vi "Parse Request-JSONtext.vi"(8 "error in (no error)":errorcluster, 10 "<JSON> Request":string) -> (0 "error out":errorcluster, 1 "params":string, 2 "method":string, 4 "id":string)   [LabVIEW 2019, in "JSON-RPC.lvlib"]
uses:
  JSON-RPC.lvlib
  66b5d778-a0b8-403e-b727-bb36a32d382a.vi
  6814ee06-2257-4c2f-8f04-31d91309bef7.vi
  f1c5ac56-d3e8-467f-aff4-e25fa4ac2541.vi
  <vilib>/JDP Science/JSONtext/JSON text to Variant.vi
  <vilib>/JDP Science/JSONtext/LVClass Serializer/JSONtext LVClass Serializer.lvclass
  <vilib>/JDP Science/JSONtext/JSONtext.lvlib
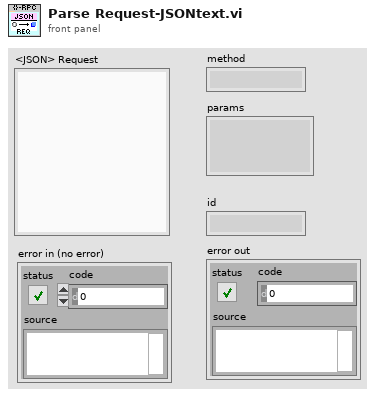
[diagram p1: front panel]
types:
  T1 = cluster{"jsconrpc":string, "method":string, "params":string, "id":string}
  T2 = enum16{"Parse Error", "Invalid Request", "Method not found", "Invalid params", "Internal error", "Server error"}
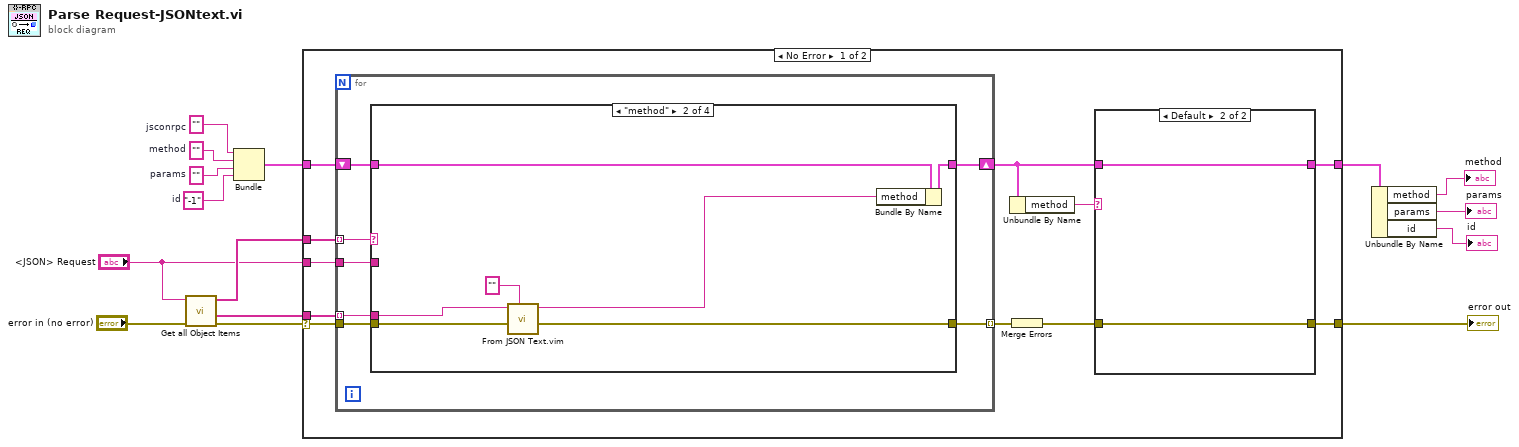
[diagram p0: block diagram]
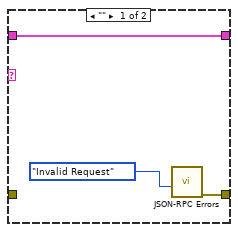
[diagram p2: hidden frame]
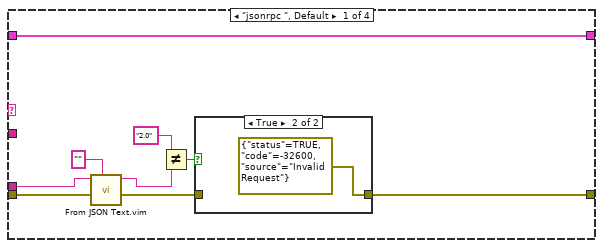
[diagram p3: hidden frame]
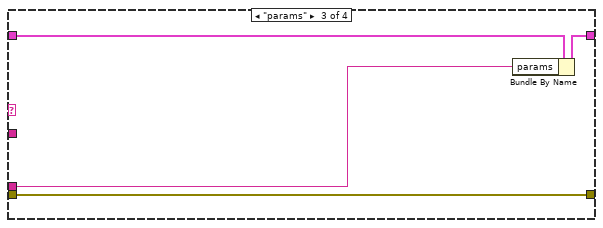
[diagram p5: hidden frame]
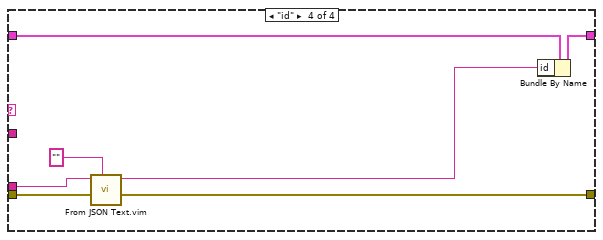
[diagram p6: hidden frame]
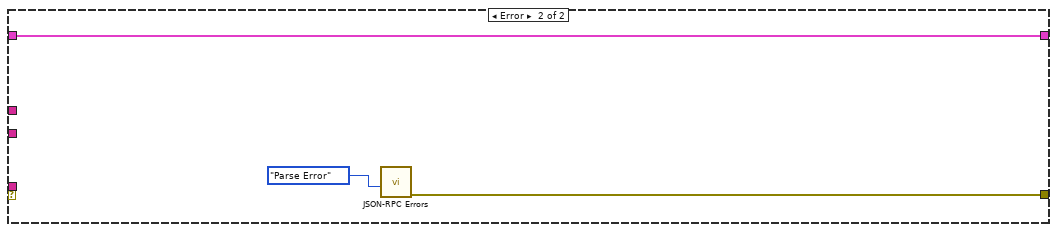
[diagram p7: hidden frame]
diagram:
  w13 = "-1"  # id
  w12 = ""  # params
  w11 = ""  # jsconrpc
  w10 = ""  # method
  n1 = call <vilib>:"Get all Object Items.vi"("error in (no error)"="error in (no error)", "JSON"="<JSON> Request") -> ("error out"=w8:errorcluster, "<JSON>"=w3:string[], "Item Names"=w9:string[])  [unwired: 6 in, 1 out]
  n2 = Bundle("jsconrpc"=w11, "method"=w10, "params"=w12, "id"=w13) -> (w14:T1)  [unwired: 1 in]
  n3 = case shown="No Error" w8 {
    selector: w8 -> [w23 _]
    tunnel: [w19 w68] -> w15
    tunnel: w14 -> [w26 w68]
    tunnel: w9 -> [w25 _]
    tunnel: [w16 w69] -> w6
    tunnel: w3 -> [w22 _]
    tunnel: "<JSON> Request" -> [w21 _]
    frame No Error {
      n4 = for {
        tunnel: w22 -> [w37] mode=indexing
        tunnel: w25 -> [w38] mode=indexing
        tunnel: w23 -> [w36]
        tunnel: [w35] -> w24 mode=indexing
        tunnel: w21 -> [w34]
        shift-right: [w32] -> w18
        shift-left: w26 -> [w33]
        n5 = case shown="\"method\"" w38 {
          tunnel: w37 -> [w40 w51 w57 w63]
          tunnel: w36 -> [w44 w56 w58 w67]
          tunnel: [w45 w55 w58 w66] -> w35
          tunnel: w34 -> [_ _ _ _]
          tunnel: w33 -> [w41 w54 w60 w65]
          tunnel: [w41 w53 w59 w64] -> w32
          frame "jsonrpc ", Default {
            n6 = call "From JSON Text.vim"("Data Type and Default Value"="", "error in (no error)"=w44, "JSON"=w40) -> ("error out"=w43:errorcluster, "Data out"=w42:string)  [unwired: 7 in]
            n7 = Not Equal?(x="2.0", y=w42) -> (x != y?=w46:bool)
            n8 = case shown="True" w46 {
              tunnel: w43 -> [w48 _]
              tunnel: [w48 errorcluster {"status"=TRUE, "code"=-32600, "source"="Invalid Request"} ("error out")] -> w45
              frame False {
              }
              frame True {
              }
            }
          }
          frame "method" {
            n9 = call "From JSON Text.vim"("Data Type and Default Value"="", "error in (no error)"=w56, "JSON"=w51) -> ("error out"=w55:errorcluster, "Data out"=w52:string)  [unwired: 7 in]
            n10 = Bundle By Name(cluster=w54, "method"=w52) -> (w53:T1)
          }
          frame "params" {
            n11 = Bundle By Name(cluster=w60, "params"=w57) -> (w59:T1)
          }
          frame "id" {
            n12 = call "From JSON Text.vim"("Data Type and Default Value"="", "error in (no error)"=w67, "JSON"=w63) -> ("error out"=w66:errorcluster, "Data out"=w61:string)  [unwired: 7 in]
            n13 = Bundle By Name(cluster=w65, "id"=w61) -> (w64:T1)
          }
        }
      }
      n14 = Unbundle By Name(w18) -> ("method"=w20:string)
      n15 = Merge Errors(w24) -> (w17:errorcluster)
      n16 = case shown="Default" w20 {
        tunnel: [w27 w31] -> w19
        tunnel: w18 -> [w27 w31]
        tunnel: w17 -> [_ w30]
        tunnel: [w28 w30] -> w16
        frame "" {
          n17 = call "JSON-RPC Errors.vi"("Enum"=T2."Invalid Request") -> ("error out"=w28:errorcluster)  [unwired: 10 in]
        }
        frame Default {
        }
      }
    }
    frame Error {
      n18 = call "JSON-RPC Errors.vi"("Enum"=T2."Parse Error") -> ("error out"=w69:errorcluster)  [unwired: 10 in]
    }
  }
  "error out" <- w6
  n19 = Unbundle By Name(w15) -> ("method"=→"method":string, "params"=→"params":string, "id"=→"id":string)
